vi "Create Client.vi"(7 "auto cleanup":bool=TRUE, 8 "error in":errorcluster, 10 "certificate path":string, 11 "address":string) -> (0 "error out":errorcluster, 3 "ClientID out":T1)   [LabVIEW 2019, in "grpc-lvsupport.lvlib"]
doc: "Creates a client that can be used to communicate with gRPC services at the specified address.\n\n<b>address</b> specifies the target address or URL of the host to connect to. \n\n<b>certificate path</b> is the file path of a certificate when making a secure connection to the target using SSL. If empty, an insecure connection is established instead.\n\n<b>auto cleanup</b> specifies if LabVIEW automatically destroys the client when the application completes execution. The default value is TRUE which means the client is automatically destroyed when the VI which created it goes idle. If <b>auto cleanup</b> is FALSE, LabVIEW does not automatically destroy the client until you exit LabVIEW or abort execution. This is useful in circumstances where you want the lifetime of the client to exceed that of the top level VI hierarchy which created it. Use <b>Close Client</b> to manually destroy the client at any time."
uses:
  grpc-lvsupport.lvlib
  Shared/grpcId.ctl
  <vilib>/Utility/error.llb/Error Cluster From Error Code.vi
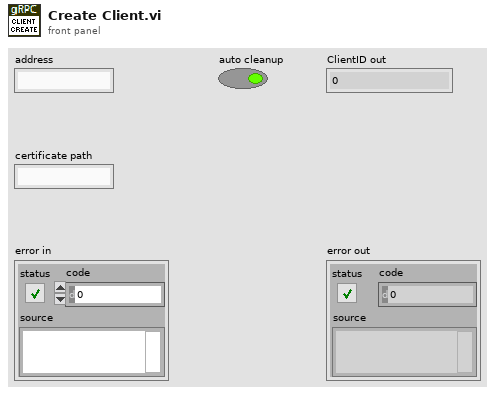
[diagram p1: front panel]
types:
  T1 = typedef "grpc-lvsupport.lvlib/grpcId.ctl" = u64
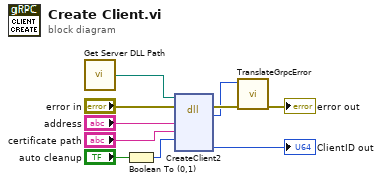
[diagram p0: block diagram]
diagram:
  n1 = call "Get Server DLL Path.vi"() -> ("Server dll path"=w8:path)
  n2 = Boolean To (0,1)(Boolean="auto cleanup") -> (0, 1=w2:i16)
  n3 = dll-call lib="?" fn="CreateClient2"(path in=w8, error in="error in", "address"="address", "certificatePath"="certificate path", "autoCleanup"=w2) -> (error out=w9:errorcluster, "return type"=w3:i32, "clientId"=→"ClientID out":u64)  [unwired: 5 in, 1 out]
  n4 = call "TranslateGrpcError.vi"("error in"=w9, "Error Code"=w3) -> ("error out"=→"error out":errorcluster)  [unwired: 9 in]
